vi "Set Up Clock Discipline.vi"(8 "error in (no error)":errorcluster, 10 "Target IP Address (empty: local)":string, 11 "RT Data Cluster in":T1={"Timekeeper hdl"="", "clkDisc session"=variant, "Compiled Data"={"SyncMod?"=FALSE, "SyncMod"="", "ConnectionSettings"={"Mode"=enum."Generate sample clock", "pxitrig"=FALSE, "pfi0"=FALSE, "pfi1"=FALSE, "pfi2"=FALSE, "External Pin"=enum."PFI0", "Routes"=[]}, "TimeKeeper"="", "ScanOffset(%)"=0.0, "StartDelay(s)"=0, "Time Ref Settings"={"Time Reference"=enum."GPS", "Priority 1"=0, "Priority 2"=0, "IRIG type"=enum."IRIGB AM", "Terminal"="", "PPSSetTime"=FALSE, "Start Time"=timestamp(0 s since 1904-01-01)}, "FIFO Locations"={"BoardTime"=[], "Status"=[]}}, "OutputsData"=[], "OutputsFIFO"=refnum, "Scan Period"=0, "Timekeeper type"=enum."6683", "SyncMod type"=enum."6683", "SyncMod hdl"="", "Custom Device Name"=""} {"Compiled Data"."Time Ref Settings"."Priority 2" min=0 max=255; "Compiled Data"."Time Ref Settings"."Priority 1" min=0 max=255}) -> (0 "error out":errorcluster, 3 "RT Data Cluster out":T1={"Timekeeper hdl"="", "clkDisc session"=variant, "Compiled Data"={"SyncMod?"=FALSE, "SyncMod"="", "ConnectionSettings"={"Mode"=enum."Generate sample clock", "pxitrig"=FALSE, "pfi0"=FALSE, "pfi1"=FALSE, "pfi2"=FALSE, "External Pin"=enum."PFI0", "Routes"=[]}, "TimeKeeper"="", "ScanOffset(%)"=0.0, "StartDelay(s)"=0, "Time Ref Settings"={"Time Reference"=enum."GPS", "Priority 1"=0, "Priority 2"=0, "IRIG type"=enum."IRIGB AM", "Terminal"="", "PPSSetTime"=FALSE, "Start Time"=timestamp(0 s since 1904-01-01)}, "FIFO Locations"={"BoardTime"=[], "Status"=[]}}, "OutputsData"=[], "OutputsFIFO"=refnum, "Scan Period"=0, "Timekeeper type"=enum."6683", "SyncMod type"=enum."6683", "SyncMod hdl"="", "Custom Device Name"=""} {"Compiled Data"."Time Ref Settings"."Priority 2" min=0 max=255; "Compiled Data"."Time Ref Settings"."Priority 1" min=0 max=255})   [LabVIEW 2020, in "NI Synchronization Engine.lvlib"]
uses:
  NI Synchronization Engine.lvlib
  RT Data Cluster.ctl
  mdevClkDisc.llb/_clkDisc_session.ctl
  Shared/Compiled Data.ctl
  Shared/Connection Settings.ctl
  Shared/Mode.ctl
  Shared/External Pin.ctl
  Shared/Routes.ctl
  Shared/Route.ctl
  Shared/Time Ref Settings.ctl
  Shared/Time Reference.ctl
  Shared/IRIG Type.ctl
  timekeeper type.ctl
  Timekeeper Route Pin.ctl
  Shared/Constants.vi
  <instrlib>/niSync/niSync.llb/niSync Initialize (Default).vi
  Shared/NI Synchronization Shared.lvlib
  System Explorer/NI Synchronization System Explorer.lvlib
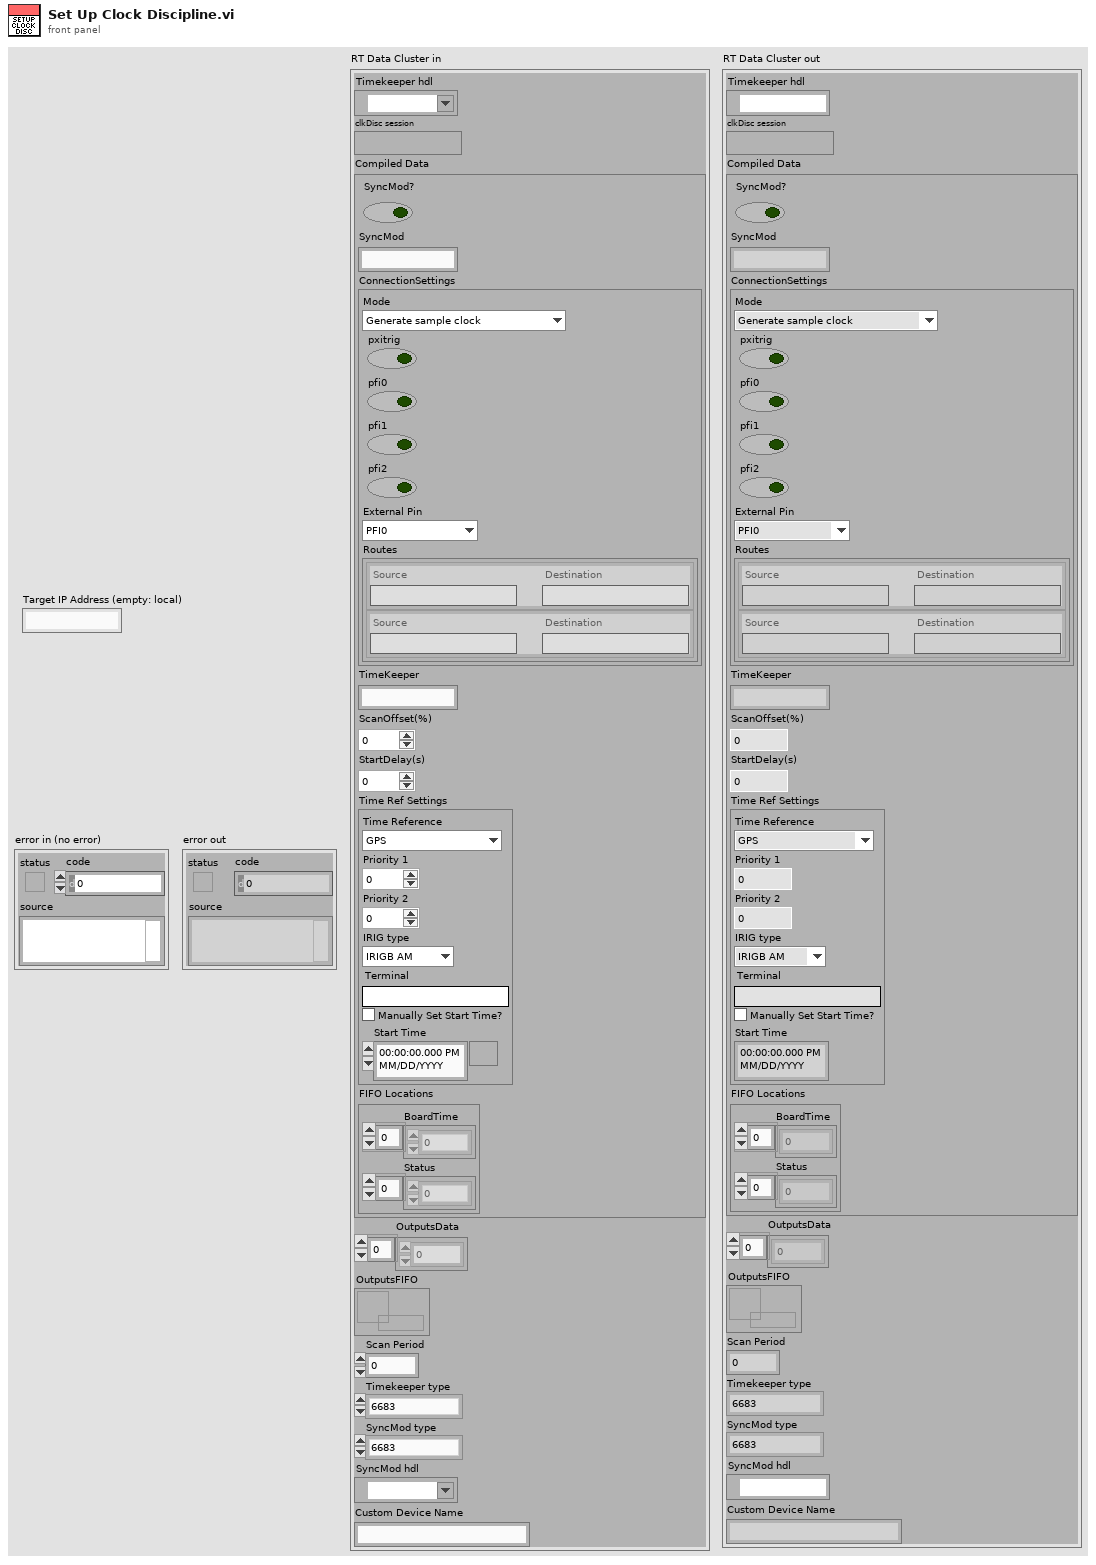
[diagram p1: front panel]
types:
  T1 = typedef "NI Synchronization Engine.lvlib/RT Data Cluster.ctl" = cluster{"Timekeeper hdl":refnum<k15>, "clkDisc session":T2, "Compiled Data":T3, "OutputsData":dbl[], "OutputsFIFO":refnum<k33>, "Scan Period":u32, "Timekeeper type":T12, "SyncMod type":T12, "SyncMod hdl":refnum<k15>, "Custom Device Name":string}
  T2 = typedef "_clkDisc_session.ctl" = variant
  T3 = typedef "NI Synchronization Shared.lvlib/Compiled Data.ctl" = cluster{"SyncMod?":bool, "SyncMod":string, "ConnectionSettings":T4, "TimeKeeper":string, "ScanOffset(%)":dbl, "StartDelay(s)":u16, "Time Ref Settings":T9, "FIFO Locations":cluster{"BoardTime":i32[], "Status":i32[]}}
  T4 = typedef "NI Synchronization Shared.lvlib/Connection Settings.ctl" = cluster{"Mode":T5, "pxitrig":bool, "pfi0":bool, "pfi1":bool, "pfi2":bool, "External Pin":T6, "Routes":T7}
  T5 = typedef "NI Synchronization Shared.lvlib/Mode.ctl" = enum16{"Generate sample clock", "Route sample clock out of chassis", "Route sample clock into chassis", "Custom routes"}
  T6 = typedef "NI Synchronization Shared.lvlib/External Pin.ctl" = enum16{"PFI0", "PFI1", "PFI2"}
  T7 = typedef "NI Synchronization Shared.lvlib/Routes.ctl" = T8[]
  T8 = typedef "NI Synchronization Shared.lvlib/Route.ctl" = cluster{"Source":string, "Destination":string}
  T9 = typedef "NI Synchronization Shared.lvlib/Time Ref Settings.ctl" = cluster{"Time Reference":T10, "Priority 1":i32, "Priority 2":i32, "IRIG type":T11, "Terminal":string, "PPSSetTime":bool, "Start Time":timestamp}
  T10 = typedef "NI Synchronization Shared.lvlib/Time Reference.ctl" = enum16{"GPS", "IRIG", "PPS", "1588 Ordinary Clock", "802.1AS", "PXI Chassis Clock", "Free Running (Internal)"}
  T11 = typedef "NI Synchronization Shared.lvlib/IRIG Type.ctl" = enum16{"IRIGB DC", "IRIGB AM"}
  T12 = typedef "NI Synchronization Engine.lvlib/timekeeper type.ctl" = enum16{"6683", "6683H", "6682", "6682H", "non-timekeeper", "timekeeper"}
  T13 = typedef "NI Synchronization Engine.lvlib/Timekeeper Route Pin.ctl" = enum16{"TTL0", "PFI0", "PFI1", "PFI2", "PXI_Clk10", "PXI_Clk10_In", "BoardClk", "ClkOut", "Oscillator"}
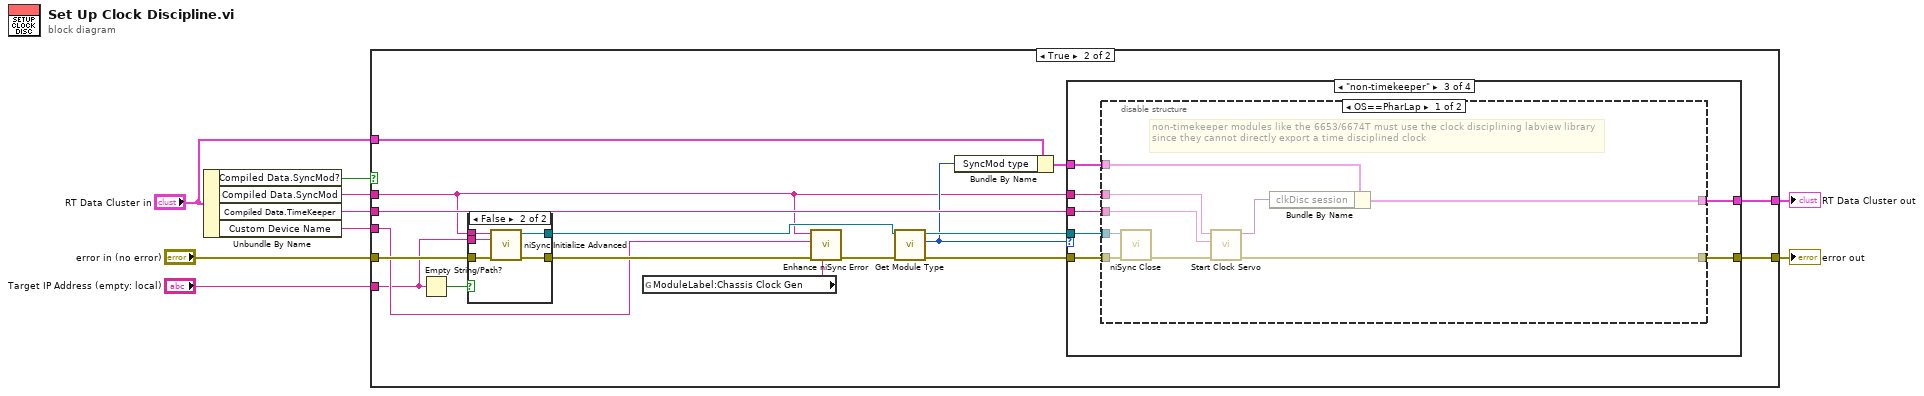
[diagram p0: block diagram]
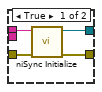
[diagram p3: hidden frame]
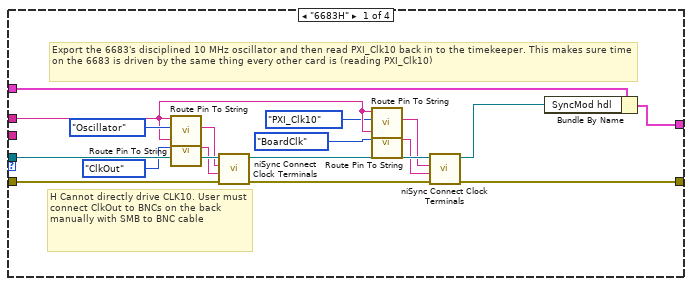
[diagram p4: hidden frame]
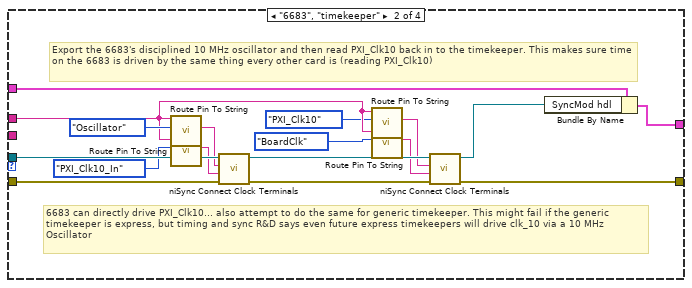
[diagram p5: hidden frame]
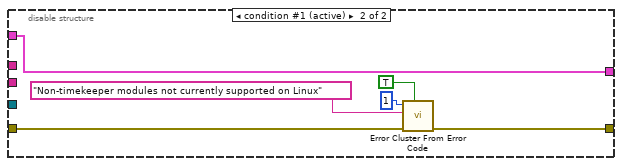
[diagram p6: hidden frame]
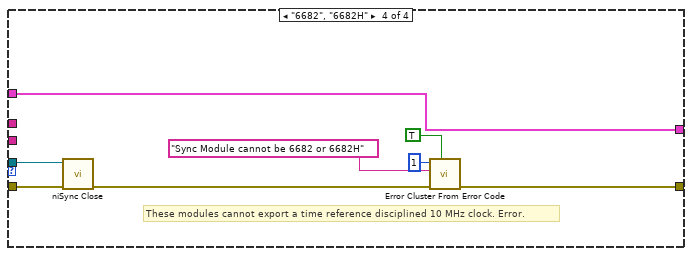
[diagram p7: hidden frame]
diagram:
  n1 = Unbundle By Name("RT Data Cluster in") -> ("Compiled Data.SyncMod?"=w9:bool, "Compiled Data.SyncMod"=w4:string, "Compiled Data.TimeKeeper"=w8:string, "Custom Device Name"=w2:string)
  n2 = case shown="True" w9 {
    tunnel: "error in (no error)" -> [w10 w23]
    tunnel: w8 -> [_ w28]
    tunnel: w4 -> [_ w16]
    tunnel: [w10 w27] -> w7
    tunnel: "RT Data Cluster in" -> [w11 w26]
    tunnel: [w11 w25] -> w5
    tunnel: w2 -> [_ w15]
    tunnel: "Target IP Address (empty: local)" -> [_ w12]
    frame False {
    }
    frame True {
      n3 = Empty String/Path?(string/path=w12) -> (empty?=w13:bool)
      n4 = case shown="False" w13 {
        tunnel: [w32 w37] -> w24
        tunnel: w23 -> [w31 w36]
        tunnel: [w30 w35] -> w18
        tunnel: w16 -> [w29 w34]
        tunnel: w12 -> [_ w33]
        frame True {
          n5 = call-poly <instrlib>:"niSync Initialize.vi"("error in (no error)"=w31, "resource name"=w29) -> ("error out"=w30:errorcluster, "instrument handle out"=w32:refnum<k15>)  [unwired: 8 in]
        }
        frame False {
          n6 = call "niSync Initialize Advanced.vi"("resource name"=w34, "remote target"=w33, "error in"=w36) -> ("instrument handle out"=w37:refnum<k15>, "error out"=w35:errorcluster)  [unwired: 11 in]
        }
      }
      n7 = global read "Constants.vi" "ModuleLabel:Chassis Clock Gen"() -> (w14:string)
      n8 = call "Enhance niSync Error.vi"("sync config label"=w14, "error in (no error)"=w18, "custom device name"=w15, "resource name"=w16) -> ("error out"=w17:errorcluster)  [unwired: 7 in]
      n9 = call "Get Module Type.vi"("error in (no error)"=w17, "IVI Refnum in"=w24) -> ("error out"=w22:errorcluster, "Module type"=w19:T12, "IVI Refnum out"=w21:refnum<k15>)  [unwired: 6 in, 1 out]
      n10 = Bundle By Name(cluster=w26, "SyncMod type"=w19) -> (w20:T1)
      n11 = case shown="\"non-timekeeper\"" w19 {
        tunnel: w28 -> [_ _ w78 _]
        tunnel: w16 -> [w40 w57 w77 _]
        tunnel: [w41 w58 w76 w100] -> w27
        tunnel: w20 -> [w54 w71 w75 w98]
        tunnel: [w51 w68 w74 w98] -> w25
        tunnel: w22 -> [w53 w70 w73 w101]
        tunnel: w21 -> [w52 w69 w72 w99]
        frame "6683H" {
          # "Export the 6683's disciplined 10 MHz oscillator and then read PXI_Clk10 back in to the timekeeper. This makes sure time on the 6683 is driven by the same thing every other card is (reading PXI_Clk10)"
          # "H Cannot directly drive CLK10. User must connect ClkOut to BNCs on the back manually with SMB to BNC cable"
          n12 = call "Route Pin To String.vi"("Pin"=Timekeeper_Route_Pin."Oscillator", "Module"=w40) -> ("String"=w50:string)  [unwired: 9 in]
          n13 = call "Route Pin To String.vi"("Pin"=Timekeeper_Route_Pin."ClkOut", "Module"=w40) -> ("String"=w49:string)  [unwired: 9 in]
          n14 = call <instrlib>:"niSync Connect Clock Terminals.vi"("error in (no error)"=w53, "destination terminal"=w49, "source terminal"=w50, "instrument handle"=w52) -> ("error out"=w45:errorcluster, "instrument handle out"=w46:refnum<k15>)  [unwired: 6 in]
          n15 = call "Route Pin To String.vi"("Pin"=Timekeeper_Route_Pin."PXI_Clk10", "Module"=w40) -> ("String"=w43:string)  [unwired: 9 in]
          n16 = call "Route Pin To String.vi"("Pin"=Timekeeper_Route_Pin."BoardClk", "Module"=w40) -> ("String"=w44:string)  [unwired: 9 in]
          n17 = call <instrlib>:"niSync Connect Clock Terminals.vi"("error in (no error)"=w45, "destination terminal"=w44, "source terminal"=w43, "instrument handle"=w46) -> ("error out"=w41:errorcluster, "instrument handle out"=w42:refnum<k15>)  [unwired: 6 in]
          n18 = Bundle By Name(cluster=w54, "SyncMod hdl"=w42) -> (w51:T1)
        }
        frame "6683", "timekeeper" {
          # "6683 can directly drive PXI_Clk10... also attempt to do the same for generic timekeeper. This might fail if the generic timekeeper is express, but timing and sync R&D says even future express timekeepers will drive clk_10 via a 10 MHz Oscillator"
          # "Export the 6683's disciplined 10 MHz oscillator and then read PXI_Clk10 back in to the timekeeper. This makes sure time on the 6683 is driven by the same thing every other card is (reading PXI_Clk10)"
          n19 = call "Route Pin To String.vi"("Pin"=Timekeeper_Route_Pin."Oscillator", "Module"=w57) -> ("String"=w67:string)  [unwired: 9 in]
          n20 = call "Route Pin To String.vi"("Pin"=Timekeeper_Route_Pin."PXI_Clk10_In", "Module"=w57) -> ("String"=w66:string)  [unwired: 9 in]
          n21 = call <instrlib>:"niSync Connect Clock Terminals.vi"("error in (no error)"=w70, "destination terminal"=w66, "source terminal"=w67, "instrument handle"=w69) -> ("error out"=w62:errorcluster, "instrument handle out"=w63:refnum<k15>)  [unwired: 6 in]
          n22 = call "Route Pin To String.vi"("Pin"=Timekeeper_Route_Pin."PXI_Clk10", "Module"=w57) -> ("String"=w60:string)  [unwired: 9 in]
          n23 = call "Route Pin To String.vi"("Pin"=Timekeeper_Route_Pin."BoardClk", "Module"=w57) -> ("String"=w61:string)  [unwired: 9 in]
          n24 = call <instrlib>:"niSync Connect Clock Terminals.vi"("error in (no error)"=w62, "destination terminal"=w61, "source terminal"=w60, "instrument handle"=w63) -> ("error out"=w58:errorcluster, "instrument handle out"=w59:refnum<k15>)  [unwired: 6 in]
          n25 = Bundle By Name(cluster=w71, "SyncMod hdl"=w59) -> (w68:T1)
        }
        frame "non-timekeeper" {
          n26 = disable-structure shown="OS==PharLap" {
            disable-tunnel: w78 -> [w87 _]
            disable-tunnel: w77 -> [w86 _]
            disable-tunnel: [w85 w88] -> w76
            disable-tunnel: w75 -> [w84 w93]
            disable-tunnel: [w83 w93] -> w74
            disable-tunnel: w73 -> [w82 w89]
            disable-tunnel: w72 -> [w81 _]
            frame condition #0 {
              # "non-timekeeper modules like the 6653/6674T must use the clock disciplining labview library since they cannot directly export a time disciplined clock"
              n27 = call <instrlib>:"niSync Close.vi"("error in (no error)"=w82, "instrument handle"=w81) -> ("error out"=w80:errorcluster)  [unwired: 9 in]
              n28 = call "Start Clock Servo.vi"("error (in)"=w80, "Time-Based Synchronization Module"=w87, "System Timing Module"=w86) -> ("error (out)"=w85:errorcluster, "clkDisc session (out)"=w79:T2)  [unwired: 3 in]
              n29 = Bundle By Name(cluster=w84, "clkDisc session"=w79) -> (w83:T1)
            }
            frame condition #1 (active) {
              n30 = call <vilib>:"Error Cluster From Error Code.vi"("show call chain? (False)"=TRUE, "error in (no error)"=w89, "error message (\"\")"="Non-timekeeper modules not currently supported on Linux" ("error message (\"\")"), "error code (0)"=1) -> ("error out"=w88:errorcluster)  [unwired: 5 in]
            }
          }
        }
        frame "6682", "6682H" {
          # "These modules cannot export a time reference disciplined 10 MHz clock. Error."
          n31 = call <instrlib>:"niSync Close.vi"("error in (no error)"=w101, "instrument handle"=w99) -> ("error out"=w94:errorcluster)  [unwired: 9 in]
          n32 = call <vilib>:"Error Cluster From Error Code.vi"("show call chain? (False)"=TRUE, "error in (no error)"=w94, "error message (\"\")"="Sync Module cannot be 6682 or 6682H" ("error message (\"\")"), "error code (0)"=1) -> ("error out"=w100:errorcluster)  [unwired: 5 in]
        }
      }
    }
  }
  "error out" <- w7
  "RT Data Cluster out" <- w5
